vi "Basler_Capture_Autocorrelator_v6.vi"() -> ()   [LabVIEW 2013]
uses:
  <vilib>/Analysis/1siggen.llb/Ramp Pattern by Samples.vi
  <vilib>/Utility/file.llb/Write To Spreadsheet File (DBL).vi
  <vilib>/Analysis/NI_AALBase.lvlib
  <vilib>/Analysis/NI_AALPro.lvlib
panel:
  in  "Image Save off":bool caption="Stop (F)"
  out "Pulse Amplitude":dbl[](array[numeric])
  out "Pulse Durations":dbl[](array[numeric])
  out "center buffer":dbl[](array[numeric])=[715.3318623600572]
  out "Now Saving":i32=119
  out "bkgnd":dbl[][](array[numeric])
  out "Save Buffer":bool
  out "T buffer":dbl[](array[numeric])=[109.07398825991858]
  out "i last":i32=118249
  in  "File Name":path=path "Autocorellator_Calibration_delay-5.82mm_n"
  in  "Stop (F) 4":bool caption="Stop (F)"
  in  "Directory":path=path "C:/Users/ut3/Desktop/JC/2011 01 24/Images"
  in  "# to save":i16=200
  in  "Stop (F) 3":bool caption="Stop (F)"
  in  "Stop (F)":bool
  in  "Tab Control":enum32{"IMAQ Image", "Intensity Graph"}(tab)=enum."Intensity Graph"
  out "Image Out":T1(plugin-control)
  out "count":i32=119
  out "i":i32=118250
  in  "History Tab":enum32{"History", "Histogram"}(tab)=enum."Histogram"
  out "Pulse dt hist.":dbl(graph)=109.07398825991858 caption="Pulse Duration history"
  in  "Save History":bool caption="Stop (F)"
  out "AC amp hist.":dbl(graph)=339.07172334171094 caption="Autocorrelation  Amplitude history"
  out "#":i64=6233
  in  "Run/Pause":bool=TRUE
  in  "Clear":bool
  in  "Save Histogram":bool
  out "Time":T2(graph)={"X Values"=[98.5926541628343, 113.97860314586778, 129.36455212890127, 144.75050111193477, 160.13645009496827, 175.52239907800177, 190.90834806103527, 206.29429704406874, 221.68024602710224, 237.06619501013574, 252.45214399316924, 267.83809297620274, 283.2240419592362, 298.6099909422697, 313.9959399253032, 329.3818889083367, 344.7678378913702, 360.1537868744037, 375.53973585743717, 390.9256848404707], "Histogram: h(x)"=[540, 2844, 2053, 539, 133, 31, 26, 16, 10, 7, 10, 3, 8, 4, 3, 2, 1, 1, 0, 2]} caption="Histogram of Pulse Durations"
  out "Time 2":T2(graph)={"X Values"=[69.1413843698024, 100.431985731182, 131.72258709256158, 163.01318845394118, 194.30378981532075, 225.59439117670036, 256.8849925380799, 288.17559389945956, 319.46619526083913, 350.7567966222187, 382.04739798359833, 413.3379993449779, 444.6286007063575, 475.9192020677371, 507.2098034291167, 538.5004047904963, 569.7910061518759, 601.0816075132554, 632.372208874635, 663.6628102360146], "Histogram: h(x)"=[12, 16, 34, 57, 208, 690, 935, 885, 812, 759, 552, 439, 254, 219, 156, 92, 55, 35, 14, 9]} caption="Histogram of Autocorrelation Amplitudes"
  in  "Calibration Tab":enum32{"Calibration", "Pulse Duration (FWHM)"}(tab)=enum."Pulse Duration (FWHM)"
  in  "x1 (pixels)":dbl=405.20982357706146
  in  "x2 (pixels)":dbl=991.9358162237035
  in  "x1 (mm)":dbl=5.79
  in  "x2 (mm)":dbl=5.85
  in  "calibrate x1":bool
  in  "calibrate x2":bool
  in  "Cal pixel/time":bool
  in  "Pixel-Time Conversion":dbl=0.6822212059025791
  out "Pulse (fs)":dbl=109.07398825991858 format="%#.3f"
  out "A.C. (pixels)":dbl=226.10542176744946
  out "Sigma center (pixels)":dbl=14.853142882292806 format="%_4f"
  out "Ave. center (pixels)":dbl=991.9358162237035 caption="center (pixels)" format="%_5f"
  in  "Sub. bkgnd":bool=TRUE caption="Stop (F)"
  in  "Save bkgnd":bool caption="Stop (F)"
  in  "Man/Auto Cursor":bool caption="Stop (F)"
  in  "AVE T":bool caption="Stop (F)"
  out "H lineout":T3(graph)
  out "V lineout":cluster{dbl[], "Ramp Pattern":dbl[]}(graph)
  out "Intensity Graph":dbl[][](graph)
  in  "Threshold Counts/Pixel":dbl=100.0 caption="Ignore Images below\nthis threshold intensity (Counts/Pixel)" format="%#.4g"
  out "Current Ave. Intensity\n(Counts/Pixel)":dbl=62.257881576038905
  in  "# to average":i32=200
  out "Sigma T (fs)":dbl=27.527803320163134 caption="Sigma" format="%_4f"
  out "Average T (fs)":dbl=147.44392289526058 caption="Average\nT (fs)" format="%_5f"
  out "Progress":i32=200
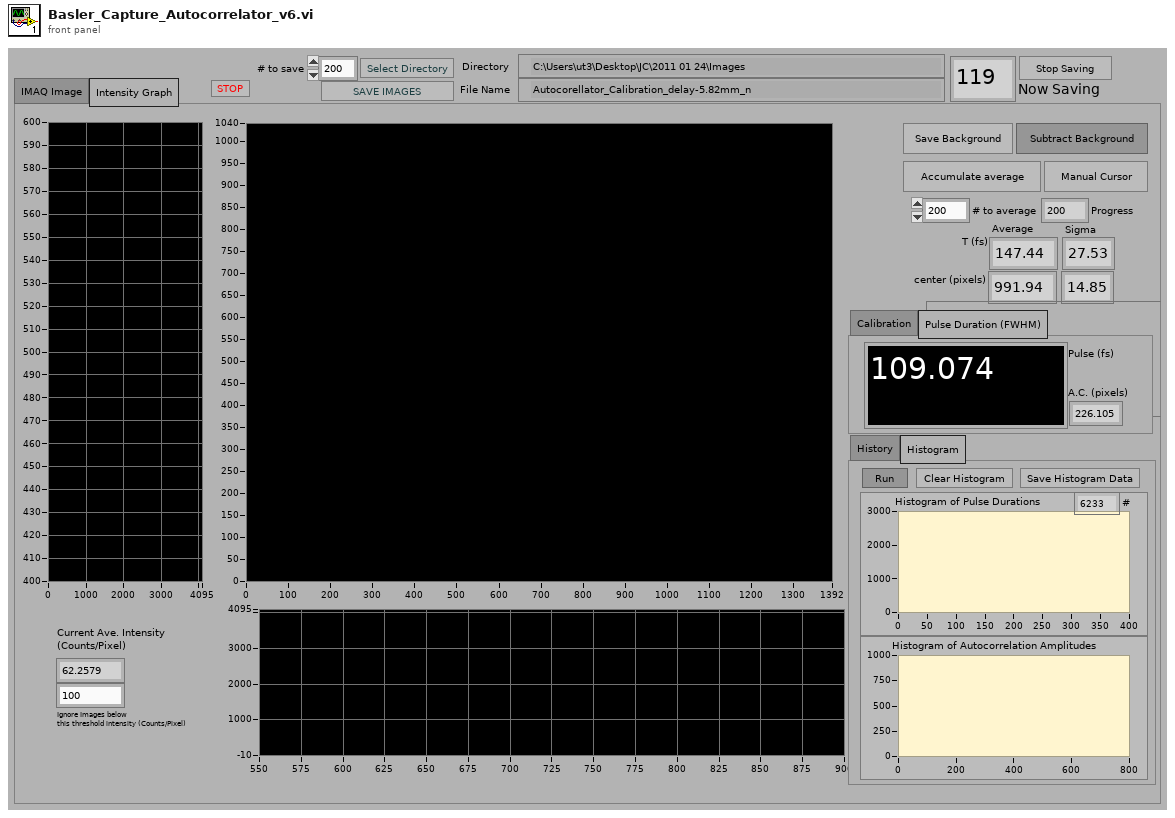
[diagram p1: front panel]
types:
  T1 = typedef "IMAQ Image.ctl" = refnum<image>
  T2 = cluster{"X Values":dbl[], "Histogram: h(x)":i32[]}
  T3 = cluster{"Ramp Pattern":dbl[], "Best Gaussian Fit":dbl[]}[]
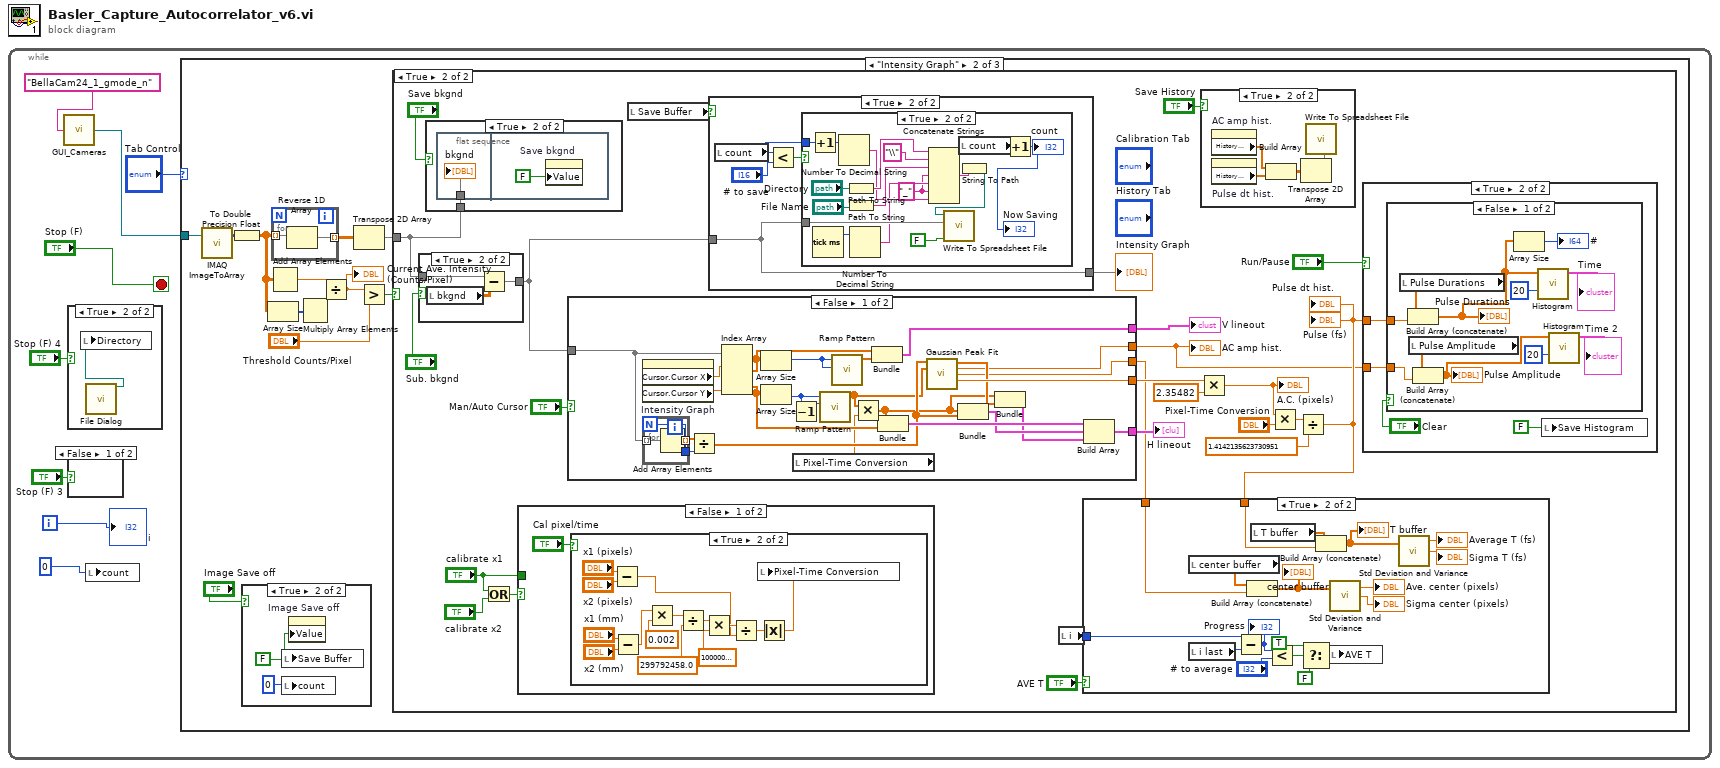
[diagram p0: block diagram]
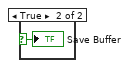
[diagram p3: hidden frame]
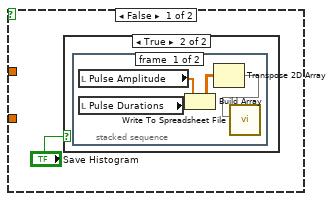
[diagram p7: hidden frame]
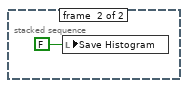
[diagram p9: hidden frame]
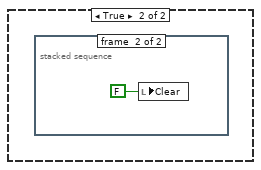
[diagram p10: hidden frame]
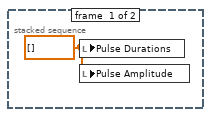
[diagram p11: hidden frame]
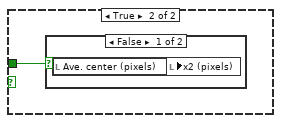
[diagram p14: hidden frame]
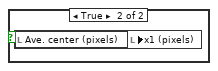
[diagram p15: hidden frame]
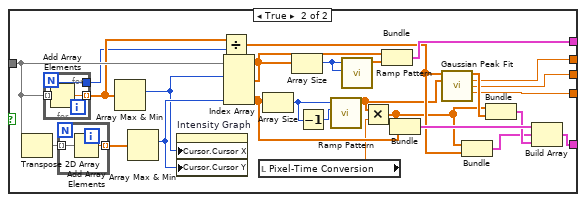
[diagram p18: hidden frame]
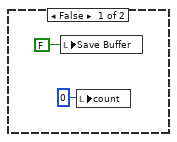
[diagram p20: hidden frame]
diagram:
  n1 = while {
    i -> [w7]
    stop <- "Stop (F)" stop-if-true
    n2 = call "GUI_Cameras.vi"("GUIdevice 1"="BellaCam24_1_gmode_n" ("GUIdevice 2")) -> ("Image (IMAQ)"=w2:T1)
    n3 = case shown="True" "Stop (F) 4" {
      frame False {
      }
      frame True {
        n4 = call "File Dialog"() -> ("selected path"=w9:path)  [unwired: 12 in, 3 out]
        n5 = local write "Directory"(w9) -> ()
      }
    }
    n6 = case shown="False" "Stop (F) 3" {
      selector: "Stop (F) 3" -> [_ w10]
      frame False {
      }
      frame True {
        "Save Buffer" <- w10
      }
    }
    n7 = local write "count"(0 ("count")) -> ()
    n8 = case shown="\"Intensity Graph\"" "Tab Control" {
      tunnel: w2 -> [_ w22 w209]
      frame Default {
      }
      frame "Intensity Graph" {
        n9 = call "IMAQ ImageToArray"("Image"=w22) -> ("Image Pixels (I16)"=w15:i16[][])  [unwired: 3 in, 4 out]
        n10 = To Double Precision Float(number=w15) -> (double precision float=w16:dbl[][])
        n11 = case shown="True" "Image Save off" {
          frame False {
          }
          frame True {
            w23 = FALSE ("Stop (F) 3")
            n12 = local write "Save Buffer"(w23) -> ()
            n13 = local write "count"(i16 0 ("#")) -> ()
            n14 = property on="Image Save off" class="Bool (strict)"("Value"=w23) -> ()  [unwired: 2 in, 2 out]
          }
        }
        n15 = Array Size(array=w16) -> (size(s)=w14:i32[])
        n16 = Add Array Elements(numeric array=w16) -> (sum=w20:dbl)
        n17 = for {
          tunnel: w16 -> [w208] mode=indexing
          tunnel: [w207] -> w17 mode=indexing
          n18 = Reverse 1D Array(array=w208) -> (reversed array=w207:dbl[])
        }
        n19 = Multiply Array Elements(1:w14) -> (0:w12:i32)
        n20 = Divide(x=w20, y=w12) -> (x/y=w19:dbl)
        "Current Ave. Intensity\n(Counts/Pixel)" <- w19
        n21 = Transpose 2D Array(2D array=w17) -> (transposed array=w18:dbl[][])
        n22 = Greater?(x=w19, y="Threshold Counts/Pixel") -> (0:w21:bool)
        n23 = case shown="True" w21 {
          tunnel: w18 -> [_ w37]
          frame False {
          }
          frame True {
            n24 = case shown="True" "Sub. bkgnd" {
              tunnel: w37 -> [w95 w97]
              tunnel: [w95 w96] -> w36
              frame False {
              }
              frame True {
                n25 = local read "bkgnd"() -> (w98:dbl[][])
                n26 = Subtract(x=w97, y=w98) -> (x-y=w96:dbl[][])
              }
            }
            n27 = case shown="True" "Save bkgnd" {
              tunnel: w37 -> [_ w99]
              frame False {
              }
              frame True {
                n28 = flat-sequence {
                  tunnel: w99 -> [w100]
                  frame #0 {
                    "bkgnd" <- w100
                  }
                  frame #1 {
                    n29 = property on="Save bkgnd" class="Bool (strict)"("Value"=FALSE ("Save bkgnd")) -> ()  [unwired: 2 in, 2 out]
                  }
                }
              }
            }
            n30 = Or(x="calibrate x1", y="calibrate x2") -> (x .or. y?=w31:bool)
            n31 = case shown="False" w31 {
              tunnel: "calibrate x1" -> [_ w92]
              frame False {
                n32 = case shown="True" "Cal pixel/time" {
                  frame False {
                  }
                  frame True {
                    n33 = Subtract(x="x1 (pixels)", y="x2 (pixels)") -> (x-y=w78:dbl)
                    n34 = Subtract(x="x1 (mm)", y="x2 (mm)") -> (x-y=w81:dbl)
                    n35 = Multiply(x=w81, y=0.002) -> (x*y=w87:dbl)
                    n36 = Divide(x=w87, y=299792458.0) -> (x/y=w85:dbl)
                    n37 = Multiply(x=w85, y=1000000000000000.0) -> (x*y=w83:dbl)
                    n38 = Divide(x=w83, y=w78) -> (x/y=w79:dbl)
                    n39 = Absolute Value(x=w79) -> (abs(x)=w86:dbl)
                    n40 = local write "Pixel-Time Conversion"(w86) -> ()
                  }
                }
              }
              frame True {
                n41 = case shown="False" w92 {
                  frame False {
                    n42 = local read "Ave. center (pixels)"() -> (w93:dbl)
                    n43 = local write "x2 (pixels)"(w93) -> ()
                  }
                  frame True {
                    n44 = local read "Ave. center (pixels)"() -> (w94:dbl)
                    n45 = local write "x1 (pixels)"(w94) -> ()
                  }
                }
              }
            }
            n46 = case shown="False" "Man/Auto Cursor" {
              tunnel: w36 -> [w113 w150]
              tunnel: [w121 w151] -> w46
              tunnel: [w118 w145] -> w45
              tunnel: [w117 w142] -> w40
              tunnel: [w109 w136] -> w26
              tunnel: [w106 w133] -> w34
              frame False {
                n47 = property on="Intensity Graph" class="IntGraph (strict)"() -> ("Cursor.Cursor X"=w124:dbl, "Cursor.Cursor Y"=w123:dbl)  [unwired: 2 in, 2 out]
                n48 = for {
                  N -> [w126]
                  tunnel: w113 -> [w128] mode=indexing
                  tunnel: [w127] -> w115 mode=indexing
                  tunnel: [w126] -> w114
                  n49 = Add Array Elements(numeric array=w128) -> (sum=w127:dbl)
                }
                n50 = Divide(x=w115, y=w114) -> (x/y=w111:dbl[])
                n51 = Index Array(array=w113, index (row) #1=w124, index (col) #2=w123) -> (element #1=w125:dbl[], element #2=w120:dbl[])  [unwired: 2 in]
                n52 = Array Size(array=w125) -> (size(s)=w122:i32)
                n53 = Array Size(array=w120) -> (size(s)=w103:i32)
                n54 = Decrement(x=w103) -> (x-1=w102:i32)
                n55 = local read "Pixel-Time Conversion"() -> (w110:dbl)
                n56 = call-poly <vilib>:"Ramp Pattern.vi"("end"=w102, "samples"=w103) -> ("Ramp Pattern"=w105:dbl[])  [unwired: 8 in, 1 out]
                n57 = call-poly <vilib>:"Ramp Pattern.vi"("end"=w122, "samples"=w122) -> ("Ramp Pattern"=w116:dbl[])  [unwired: 8 in, 1 out]
                n58 = Multiply(x=w105, y=w110) -> (x*y=w104:dbl[])
                n59 = Bundle(w125, "Ramp Pattern"=w116) -> (w121:cluster{dbl[], "Ramp Pattern":dbl[]})  [unwired: 1 in]
                n60 = Bundle(w104, w120) -> (w119:cluster{dbl[], dbl[]})  [unwired: 1 in]
                n61 = call <vilib>:"Gaussian Peak Fit.vi"("Y"=w111, "X"=w105) -> ("Best Gaussian Fit"=w112:dbl[], "amplitude"=w109:dbl, "center"=w106:dbl, "standard deviation"=w117:dbl)  [unwired: 7 in, 3 out]
                n62 = Bundle(w104, w111) -> (w108:cluster{dbl[], dbl[]})  [unwired: 1 in]
                n63 = Bundle(w104, "Best Gaussian Fit"=w112) -> (w107:cluster{dbl[], "Best Gaussian Fit":dbl[]})  [unwired: 1 in]
                n64 = Build Array(w119, w108, w107) -> (w118:cluster{dbl[], "Best Gaussian Fit":dbl[]}[])
              }
              frame True {
                n65 = Transpose 2D Array(2D array=w150) -> (transposed array=w149:dbl[][])
                n66 = for {
                  N -> [w157]
                  tunnel: w150 -> [w159] mode=indexing
                  tunnel: [w158] -> w139 mode=indexing
                  tunnel: [w157] -> w138
                  n67 = Add Array Elements(numeric array=w159) -> (sum=w158:dbl)
                }
                n68 = for {
                  tunnel: w149 -> [w156] mode=indexing
                  tunnel: [w155] -> w141 mode=indexing
                  n69 = Add Array Elements(numeric array=w156) -> (sum=w155:dbl)
                }
                n70 = Array Max & Min(array=w139) -> (max index (indices)=w140:i32)  [unwired: 3 out]
                n71 = Array Max & Min(array=w141) -> (max index (indices)=w148:i32)  [unwired: 3 out]
                n72 = property on="Intensity Graph" class="IntGraph (strict)"("Cursor.Cursor X"=w140, "Cursor.Cursor Y"=w148) -> ()  [unwired: 2 in, 2 out]
                n73 = Divide(x=w139, y=w138) -> (x/y=w135:dbl[])
                n74 = Index Array(array=w150, index (row) #1=w140, index (col) #2=w148) -> (element #1=w154:dbl[], element #2=w147:dbl[])  [unwired: 2 in]
                n75 = local read "Pixel-Time Conversion"() -> (w137:dbl)
                n76 = Array Size(array=w147) -> (size(s)=w129:i32)
                n77 = Array Size(array=w154) -> (size(s)=w152:i32)
                n78 = Decrement(x=w129) -> (x-1=w130:i32)
                n79 = call-poly <vilib>:"Ramp Pattern.vi"("end"=w130, "samples"=w129) -> ("Ramp Pattern"=w132:dbl[])  [unwired: 8 in, 1 out]
                n80 = call-poly <vilib>:"Ramp Pattern.vi"("end"=w152, "samples"=w152) -> ("Ramp Pattern"=w153:dbl[])  [unwired: 8 in, 1 out]
                n81 = Multiply(x=w132, y=w137) -> (x*y=w131:dbl[])
                n82 = Bundle(w154, "Ramp Pattern"=w153) -> (w151:cluster{dbl[], "Ramp Pattern":dbl[]})  [unwired: 1 in]
                n83 = Bundle(w131, w147) -> (w146:cluster{dbl[], dbl[]})  [unwired: 1 in]
                n84 = call <vilib>:"Gaussian Peak Fit.vi"("Y"=w135, "X"=w132) -> ("Best Gaussian Fit"=w143:dbl[], "amplitude"=w136:dbl, "center"=w133:dbl, "standard deviation"=w142:dbl)  [unwired: 7 in, 3 out]
                n85 = Bundle(w131, w135) -> (w134:cluster{dbl[], dbl[]})  [unwired: 1 in]
                n86 = Bundle(w131, "Best Gaussian Fit"=w143) -> (w144:cluster{dbl[], "Best Gaussian Fit":dbl[]})  [unwired: 1 in]
                n87 = Build Array(w146, w134, w144) -> (w145:cluster{dbl[], "Best Gaussian Fit":dbl[]}[])
              }
            }
            "V lineout" <- w46
            "H lineout" <- w45
            "AC amp hist." <- w26
            n88 = local read "Save Buffer"() -> (w47:bool)
            n89 = case shown="True" w47 {
              tunnel: w36 -> [w160 w161]
              tunnel: [w160 w161] -> w33
              frame False {
              }
              frame True {
                n90 = local read "count"() -> (w162:i32)
                n91 = Less?(x=w162, y="# to save") -> (x < y?=w163:bool)
                n92 = case shown="True" w163 {
                  tunnel: w161 -> [_ w183]
                  tunnel: w162 -> [_ w182]
                  frame False {
                    n93 = local write "Save Buffer"(FALSE ("Stop (F) 3")) -> ()
                    n94 = local write "count"(i16 0 ("#")) -> ()
                  }
                  frame True {
                    w169 = "_" ("string")
                    n95 = Increment(x=w182) -> (x+1=w178:i32)
                    n96 = Tick Count (ms)() -> (millisecond timer value=w172:u32)
                    n97 = Number To Decimal String(number=w178) -> (decimal integer string=w171:string)  [unwired: 1 in]
                    n98 = Path To String(path="Directory") -> (string=w181:string)
                    n99 = Path To String(path="File Name") -> (string=w173:string)
                    n100 = Number To Decimal String(number=w172) -> (decimal integer string=w170:string)  [unwired: 1 in]
                    n101 = Concatenate Strings(w181, "\\" ("string"), w173, w169, w170, w169, w171) -> (w180:string)
                    n102 = local read "count"() -> (w168:i32)
                    n103 = String To Path(string=w180) -> (path=w179:path)
                    n104 = call-poly <vilib>:"Write To Spreadsheet File.vi"("append to file? (new file:F)"=FALSE, "2D data"=w183, "file path (dialog if empty)"=w179) -> ()  [unwired: 5 in, 1 out]
                    n105 = Increment(x=w168) -> (x+1=→"count" →"Now Saving":i32)
                  }
                }
              }
            }
            "Intensity Graph" <- w33
            n106 = local read "i"() -> (w48:i32)
            n107 = Multiply(x=w40, y=2.35482) -> (x*y=w42:dbl)
            "A.C. (pixels)" <- w42
            n108 = case shown="True" "Save History" {
              frame False {
              }
              frame True {
                n109 = property on="AC amp hist." class="WFChart (strict)"() -> ("History Data"=w76:dbl[])  [unwired: 2 in, 2 out]
                n110 = property on="Pulse dt hist." class="WFChart (strict)"() -> ("History Data"=w75:dbl[])  [unwired: 2 in, 2 out]
                n111 = Build Array(w76, w75) -> (w74:dbl[][])
                n112 = Transpose 2D Array(2D array=w74) -> (transposed array=w73:dbl[][])
                n113 = call-poly <vilib>:"Write To Spreadsheet File.vi"("2D data"=w73) -> ()  [unwired: 7 in, 1 out]
              }
            }
            n114 = Multiply(x=w42, y="Pixel-Time Conversion") -> (x*y=w35:dbl)
            n115 = Divide(x=w35, y=1.4142135623730951) -> (x/y=w27:dbl)
            "Pulse (fs)" <- w27
            "Pulse dt hist." <- w27
            n116 = case shown="True" "AVE T" {
              tunnel: w27 -> [w187 w198]
              tunnel: w48 -> [w188 w206]
              tunnel: w34 -> [w185 w191]
              frame False {
                n117 = Build Array(w185) -> (w184:dbl[])
                n118 = local write "center buffer"(w184) -> ()
                n119 = Build Array(w187) -> (w186:dbl[])
                n120 = local write "T buffer"(w186) -> ()
                "i last" <- w188
              }
              frame True {
                n121 = local read "center buffer"() -> (w189:dbl[])
                n122 = local read "i last"() -> (w205:i32)
                n123 = Subtract(x=w206, y=w205) -> (x-y=w199:i32)
                "Progress" <- w199
                n124 = Build Array (concatenate)(w189, w191) -> (w190:dbl[])
                "center buffer" <- w190
                n125 = local read "T buffer"() -> (w197:dbl[])
                n126 = Less?(x=w199, y="# to average") -> (x < y?=w203:bool)
                n127 = Select(t=TRUE, s=w203, f=FALSE) -> (s? t:f=w202:bool)
                n128 = Build Array (concatenate)(w197, w198) -> (w196:dbl[])
                "T buffer" <- w196
                n129 = local write "AVE T"(w202) -> ()
                n130 = call <vilib>:"Std Deviation and Variance.vi"("X"=w190) -> ("mean"=→"Ave. center (pixels)":dbl, "standard deviation"=→"Sigma center (pixels)":dbl)  [unwired: 1 in, 1 out]
                n131 = call <vilib>:"Std Deviation and Variance.vi"("X"=w196) -> ("mean"=→"Average T (fs)":dbl, "standard deviation"=→"Sigma T (fs)":dbl)  [unwired: 1 in, 1 out]
              }
            }
            n132 = case shown="True" "Run/Pause" {
              tunnel: w27 -> [_ w59]
              tunnel: w26 -> [_ w58]
              frame False {
                n133 = case shown="True" "Save Histogram" {
                  frame False {
                  }
                  frame True {
                    n134 = stacked-sequence {
                      frame #0 {
                        n135 = local read "Pulse Amplitude"() -> (w53:dbl[])
                        n136 = local read "Pulse Durations"() -> (w54:dbl[])
                        n137 = Build Array(w53, w54) -> (w52:dbl[][])
                        n138 = Transpose 2D Array(2D array=w52) -> (transposed array=w51:dbl[][])
                        n139 = call-poly <vilib>:"Write To Spreadsheet File.vi"("2D data"=w51) -> ()  [unwired: 7 in, 1 out]
                      }
                      frame #1 {
                        n140 = local write "Save Histogram"(FALSE ("Save Histogram")) -> ()
                      }
                    }
                  }
                }
              }
              frame True {
                n141 = case shown="False" "Clear" {
                  tunnel: w59 -> [w69 _]
                  tunnel: w58 -> [w68 _]
                  frame False {
                    n142 = local read "Pulse Durations"() -> (w70:dbl[])
                    n143 = Build Array (concatenate)(w70, w69) -> (w61:dbl[])
                    "Pulse Durations" <- w61
                    n144 = local read "Pulse Amplitude"() -> (w67:dbl[])
                    n145 = Build Array (concatenate)(w67, w68) -> (w62:dbl[])
                    "Pulse Amplitude" <- w62
                    n146 = Array Size(array=w61) -> (size(s)=→"#":i32)
                    n147 = call <vilib>:"Histogram.vi"("intervals"=20, "X"=w61) -> ("Histogram Graph"=→"Time":T2)  [unwired: 6 in, 3 out]
                    n148 = call <vilib>:"Histogram.vi"("intervals"=20, "X"=w62) -> ("Histogram Graph"=→"Time 2":T2)  [unwired: 6 in, 3 out]
                  }
                  frame True {
                    n149 = stacked-sequence {
                      frame #0 {
                        w71 = dbl[] [] ("Pulse Durations")
                        n150 = local write "Pulse Durations"(w71) -> ()
                        n151 = local write "Pulse Amplitude"(w71) -> ()
                      }
                      frame #1 {
                        n152 = local write "Clear"(FALSE ("Clear")) -> ()
                      }
                    }
                  }
                }
                n153 = local write "Save Histogram"(FALSE ("Save Histogram")) -> ()
              }
            }
          }
        }
      }
      frame "IMAQ Image" {
        "Image Out" <- w209
      }
    }
    "i" <- w7
  }
